vi "Read Help Info File.vi"(8 "error in":errorcluster, 11 "Help Info File":path) -> (0 "error out":errorcluster, 1 "Help Items":T1(array[cluster]), 2 "Help Paths":T2, 3 "dup Help Info File":path)   [LabVIEW 2014, in "VIHelpeksAPI.lvlib"]
doc: "The VI reads the <b>Help Info File</b> generated by VI Helpeks during help generation. The <b>Help Info File</b> contains information about the source VIs, their respective HTML files, and the information required for linking them. It also indicates details on .HHP and .CHM files if any were generated.\n\nThe <b>Example VI</b> demonstrating the use of VIHelpeks API can be opened using the \"Tools >> VI Helpeks >> Help and Support\" menu. Alternatively, you can launch the <b>NI Example Finder</b> and search for \"VI Helpeks\", or find it within the <b><labview>\\Examples\\VI Helpeks</b> folder.\n\n::: VI Helpeks :::\nCopyright (c) 2000-2026 Konstantin Shifershteyn. All rights reserved."
uses:
  VIHelpeksAPI.lvlib
  <vilib>/Utility/config.llb/Read Key (Path).vi
  <vilib>/Utility/config.llb/Read Key (String).vi
  <vilib>/Utility/config.llb/NI_LVConfig.lvlib
panel:
  # "VI Helpeks\nCopyright (c) 2012-2026 Konstantin Shifershteyn"
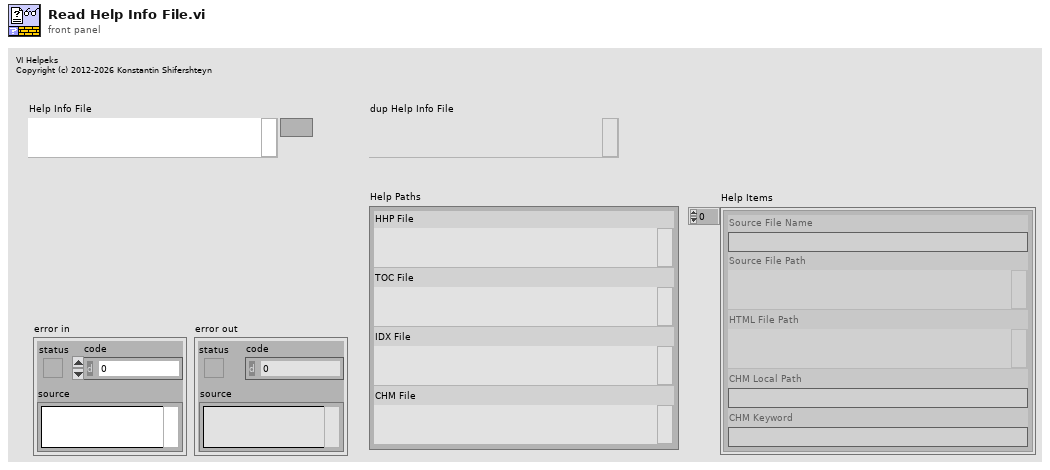
[diagram p1: front panel]
types:
  T1 = cluster{"Source File Name":string, "Source File Path":path, "HTML File Path":path, "CHM Local Path":string, "CHM Keyword":string}[]
  T2 = cluster{"HHP File":path, "TOC File":path, "IDX File":path, "CHM File":path}
  T3 = typedef "NI_LVConfig.lvlib/Config Data RefNum.ctl" = refnum<k1>
  T4 = cluster{"value":string, "value":path, "value":path, "value":string, "value":string}
  T5 = cluster{"[0]":path, "[1]":path, "[2]":path, "[3]":path}
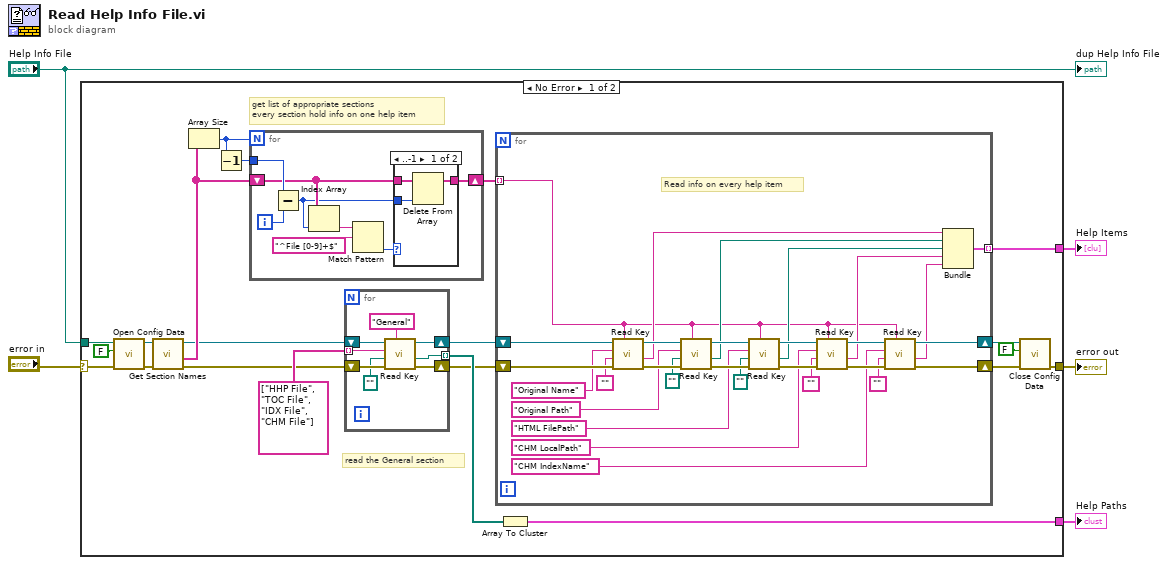
[diagram p0: block diagram]
diagram:
  n1 = case shown="No Error" "error in" {
    selector: "error in" -> [w6 w76]
    tunnel: [w23 _] -> w5
    tunnel: [w22 _] -> w4
    tunnel: [w18 w76] -> w3
    tunnel: "Help Info File" -> [w7 _]
    frame No Error {
      # "read the General section"
      # "get list of appropriate sections\nevery section hold info on one help item"
      n2 = call <vilib>:"Open Config Data.vi"("error in (no error)"=w6, "create file if necessary (T)"=FALSE, "configuration file path"=w7) -> ("error out"=w11:errorcluster, "refnum"=w12:T3)  [unwired: 6 in, 1 out]
      n3 = call <vilib>:"Get Section Names.vi"("error in (no error)"=w11, "refnum"=w12) -> ("error out"=w9:errorcluster, "section names"=w15:string[], "refnum out"=w10:T3)  [unwired: 7 in]
      n4 = Array Size(array=w15) -> (size(s)=w16:i32)
      n5 = Decrement(x=w16) -> (x-1=w17:i32)
      n6 = for {
        N: w16 -> [_]
        shift-right: [w31] -> w8
        shift-left: w15 -> [w32]
        tunnel: w17 -> [w33]
        i -> [w34]
        n7 = Subtract(x=w33, y=w34) -> (x-y=w30:i32)
        n8 = Index Array(array=w32, index=w30) -> (element=w29:string)
        n9 = Match Pattern(string=w29, regular expression="^File [0-9]+$") -> (offset past match=w28:i32)  [unwired: 1 in, 3 out]
        n10 = case shown="..-1" w28 {
          tunnel: w32 -> [w37 w38]
          tunnel: [w36 w38] -> w31
          tunnel: w30 -> [w35 _]
          frame ..-1 {
            n11 = Delete From Array(array=w37, index=w35) -> (array with subset deleted=w36:string[])  [unwired: 1 in, 1 out]
          }
          frame 0.. {
          }
        }
      }
      n12 = for {
        tunnel: string[] ["HHP File", "TOC File", "IDX File", "CHM File"] -> [w71] mode=indexing
        shift-right: [w70] -> w14
        shift-left: w10 -> [w75]
        shift-right: [w69] -> w13
        shift-left: w9 -> [w74]
        tunnel: [w68] -> w24 mode=indexing
        n13 = call-poly <vilib>:"Read Key.vi"("section"="General", "error in (no error)"=w74, "default value"=path "", "key"=w71, "refnum"=w75) -> ("error out"=w69:errorcluster, "value"=w68:path, "refnum out"=w70:T3)  [unwired: 3 in, 1 out]
      }
      n14 = for {
        shift-right: [w47] -> w21
        shift-left: w14 -> [w67]
        shift-right: [w46] -> w19
        shift-left: w13 -> [w66]
        tunnel: [w40] -> w22 mode=indexing
        tunnel: w8 -> [w39] mode=indexing
        # "Read info on every help item"
        n15 = call-poly <vilib>:"Read Key.vi"("section"=w39, "error in (no error)"=w66, "default value"="", "key"="Original Name", "refnum"=w67) -> ("error out"=w61:errorcluster, "value"=w45:string, "refnum out"=w65:T3)  [unwired: 3 in, 1 out]
        n16 = call-poly <vilib>:"Read Key.vi"("section"=w39, "error in (no error)"=w61, "default value"=path "", "key"="Original Path", "refnum"=w65) -> ("error out"=w60:errorcluster, "value"=w44:path, "refnum out"=w64:T3)  [unwired: 3 in, 1 out]
        n17 = call-poly <vilib>:"Read Key.vi"("section"=w39, "error in (no error)"=w60, "default value"=path "", "key"="HTML FilePath", "refnum"=w64) -> ("error out"=w59:errorcluster, "value"=w43:path, "refnum out"=w63:T3)  [unwired: 3 in, 1 out]
        n18 = call-poly <vilib>:"Read Key.vi"("section"=w39, "error in (no error)"=w59, "default value"="", "key"="CHM LocalPath", "refnum"=w63) -> ("error out"=w58:errorcluster, "value"=w42:string, "refnum out"=w62:T3)  [unwired: 3 in, 1 out]
        n19 = call-poly <vilib>:"Read Key.vi"("section"=w39, "error in (no error)"=w58, "default value"="", "key"="CHM IndexName", "refnum"=w62) -> ("error out"=w46:errorcluster, "value"=w41:string, "refnum out"=w47:T3)  [unwired: 3 in, 1 out]
        n20 = Bundle("value"=w45, "value"=w44, "value"=w43, "value"=w42, "value"=w41) -> (w40:T4)  [unwired: 1 in]
      }
      n21 = Array To Cluster(array=w24) -> (cluster=w23:T5)
      n22 = call <vilib>:"Close Config Data.vi"("error in (no error)"=w19, "write file if changed (T)"=FALSE, "refnum"=w21) -> ("error out"=w18:errorcluster)  [unwired: 7 in, 1 out]
    }
    frame Error {
    }
  }
  "error out" <- w3
  "Help Paths" <- w5
  "Help Items" <- w4
  "dup Help Info File" <- "Help Info File"
